vi "Delte-table.vi"(10 "Indix":i32=3, 11 "数组":string[][](array[string])=[["1", "3"], ["2", "4"], ["新建表1", ""]]) -> (2 "Old-table":string, 3 "输出数组":string[][](array[string]))   [LabVIEW 2025]
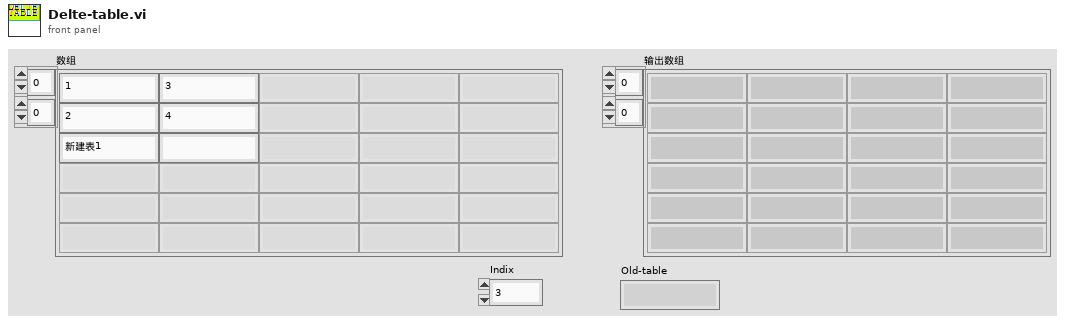
[diagram p1: front panel]
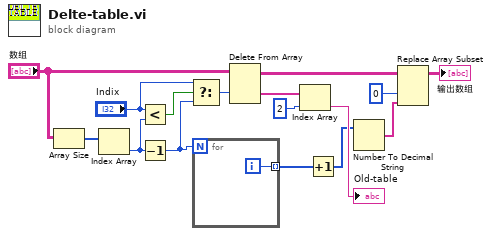
[diagram p0: block diagram]
diagram:
  n1 = Array Size(array="数组") -> (size(s)=w12:i32[])
  n2 = Index Array(array=w12) -> (element=w4:i32)  [unwired: 1 in]
  n3 = Less?(x="Indix", y=w4) -> (x < y?=w11:bool)
  n4 = Decrement(x=w4) -> (x-1=w1:i32)
  n5 = Select(t="Indix", s=w11, f=w1) -> (s? t:f=w9:i32)
  n6 = for {
    N: w1 -> [_]
    tunnel: [w17] -> w6 mode=indexing
    i -> [w17]
  }
  n7 = Delete From Array(array="数组", index (row)=w9) -> (deleted portion=w16:string[], array with subset deleted=w8:string[][])  [unwired: 2 in]
  n8 = Index Array(array=w16, index=2 ("索引")) -> (element=→"Old-table":string)
  n9 = Increment(x=w6) -> (x+1=w5:i32[])
  n10 = Number To Decimal String(number=w5) -> (decimal integer string=w3:string[])  [unwired: 1 in]
  n11 = Replace Array Subset(array=w8, new element=w3, index (col)=0 ("禁用的索引 (列)")) -> (→"输出数组":string[][])  [unwired: 1 in]
